vi "Sim_Update_Model.vi"(8 "dt (s)":dbl, 9 "State":T3, 10 "Settings":T4={"UI Update Interval (ms)"=200, "Max dt (s)"=1.0, "Initial SOC (%)"=50.0, "Rest Voltage (V)"=12.0, "Ambient Temperature (degC)"=25.0, "Voltage Time Constant (s)"=5.0, "Current Time Constant (s)"=1.0, "Thermal Time Constant (s)"=120.0, "Heating Coefficient (degC/s per A^2)"=0.002, "SOC Speed Factor"=1.0, "Charge Complete SOC (%)"=100.0, "Discharge Complete SOC (%)"=0.0, "Max Voltage Limit (V)"=15.0, "Max Current Limit (A)"=10.0, "Max Temperature Limit (degC)"=45.0, "Max C-Rate (1/h)"=5.0, "Max Duration (min)"=600.0, "History Length (samples)"=3000, "Inject E-Stop"=FALSE, "Inject Overvoltage"=FALSE, "Inject Overcurrent"=FALSE, "Inject Overtemperature"=FALSE}, 11 "Sim Data in":T1) -> (3 "Sim Data out":T1)   [LabVIEW 2019]
doc: "DEMONSTRATION MODEL - the replaceable sensor source. One simulation step of length dt. SOC: ideal C-rate integration (dSOC = C x 100 x dt x SpeedFactor / 3600) clamped 0..100. Voltage and current: first-order approach to the setpoints (discharge current negative). Temperature: current-squared heating with first-order cooling to ambient. OUTPUT INTERLOCK: only CHARGING enables the simulated supply and only DISCHARGING the simulated load; every other state forces both OFF and current to 0. Not an electrochemical battery model. A later hardware phase replaces this VI."
uses:
  Sim_Data.ctl
  Test_State_Enum2.ctl
  Sim_Settings.ctl
  Sim_State_Enum.ctl
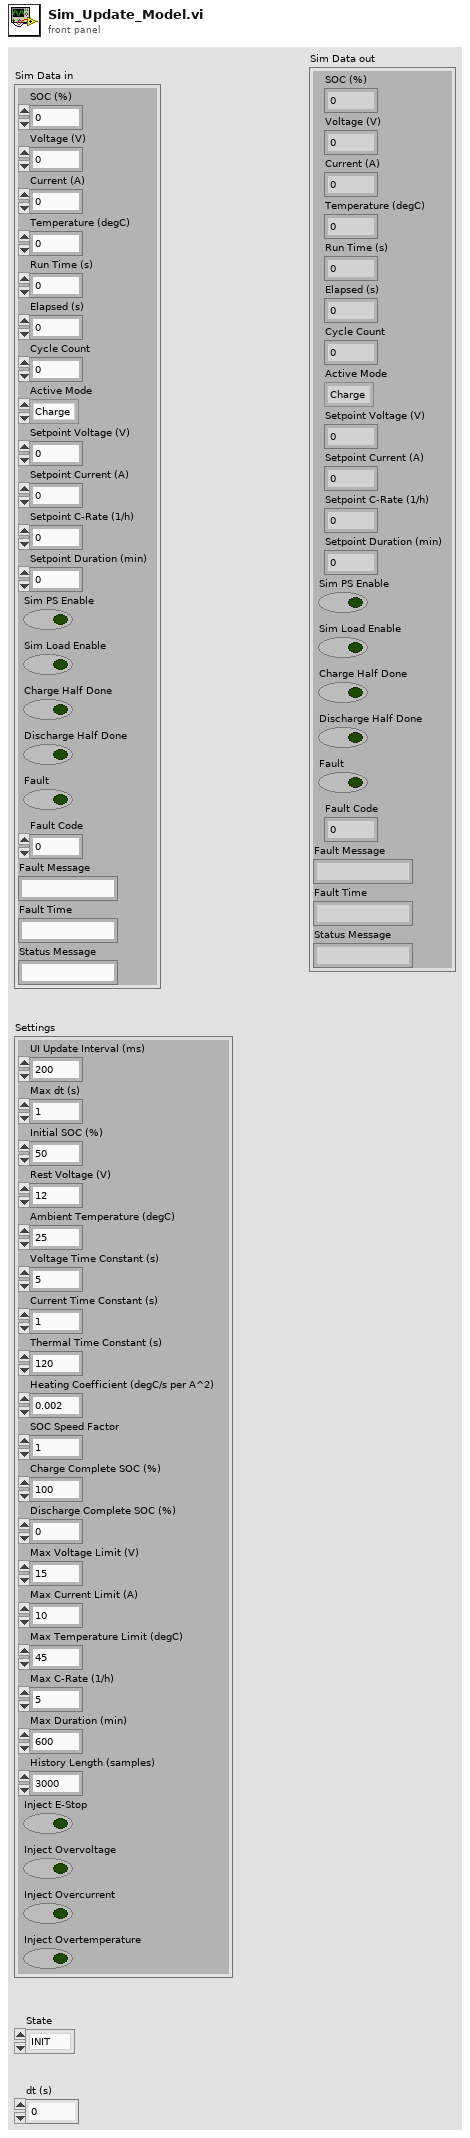
[diagram p1: front panel]
types:
  T1 = typedef "Sim_Data.ctl" = cluster{"SOC (%)":dbl, "Voltage (V)":dbl, "Current (A)":dbl, "Temperature (degC)":dbl, "Run Time (s)":dbl, "Elapsed (s)":dbl, "Cycle Count":u32, "Active Mode":T2, "Setpoint Voltage (V)":dbl, "Setpoint Current (A)":dbl, "Setpoint C-Rate (1/h)":dbl, "Setpoint Duration (min)":dbl, "Sim PS Enable":bool, "Sim Load Enable":bool, "Charge Half Done":bool, "Discharge Half Done":bool, "Fault":bool, "Fault Code":i32, "Fault Message":string, "Fault Time":string, "Status Message":string}
  T2 = typedef "Test_State_Enum2.ctl" = enum16{"Charge", "Discharge"}
  T3 = typedef "Sim_State_Enum.ctl" = enum16{"INIT", "IDLE", "CHARGING", "DISCHARGING", "STOPPED", "FAULT"}
  T4 = typedef "Sim_Settings.ctl" = cluster{"UI Update Interval (ms)":i32, "Max dt (s)":dbl, "Initial SOC (%)":dbl, "Rest Voltage (V)":dbl, "Ambient Temperature (degC)":dbl, "Voltage Time Constant (s)":dbl, "Current Time Constant (s)":dbl, "Thermal Time Constant (s)":dbl, "Heating Coefficient (degC/s per A^2)":dbl, "SOC Speed Factor":dbl, "Charge Complete SOC (%)":dbl, "Discharge Complete SOC (%)":dbl, "Max Voltage Limit (V)":dbl, "Max Current Limit (A)":dbl, "Max Temperature Limit (degC)":dbl, "Max C-Rate (1/h)":dbl, "Max Duration (min)":dbl, "History Length (samples)":i32, "Inject E-Stop":bool, "Inject Overvoltage":bool, "Inject Overcurrent":bool, "Inject Overtemperature":bool}
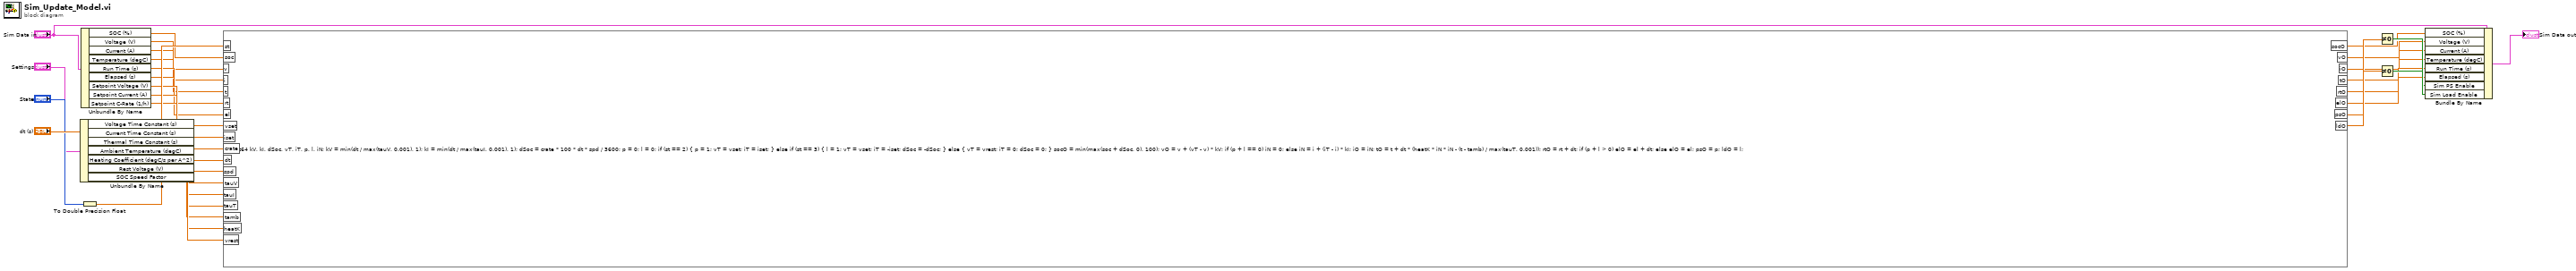
[diagram p0: block diagram]
diagram:
  n1 = Unbundle By Name("Settings") -> ("Voltage Time Constant (s)"=w15:dbl, "Current Time Constant (s)"=w16:dbl, "Thermal Time Constant (s)"=w17:dbl, "Ambient Temperature (degC)"=w18:dbl, "Heating Coefficient (degC/s per A^2)"=w19:dbl, "Rest Voltage (V)"=w20:dbl, "SOC Speed Factor"=w21:dbl)
  n2 = Unbundle By Name("Sim Data in") -> ("SOC (%)"=w6:dbl, "Voltage (V)"=w7:dbl, "Current (A)"=w8:dbl, "Temperature (degC)"=w9:dbl, "Run Time (s)"=w10:dbl, "Elapsed (s)"=w11:dbl, "Setpoint Voltage (V)"=w12:dbl, "Setpoint Current (A)"=w13:dbl, "Setpoint C-Rate (1/h)"=w14:dbl)
  n3 = To Double Precision Float(number="State") -> (double precision float=w22:dbl)
  n4 = formula code="float64 kV, kI, dSoc, vT, iT, p, l, iN; kV = min(dt / max(tauV, 0.001), 1); kI = min(dt / max(tauI, 0.001), 1); dSoc = crate * 100 * dt * spd / 3600; p = 0; l = 0; if (st == 2) { p = 1; vT = vset; iT = iset; } else if (st == 3) { l = 1; vT = vset; iT = -iset; dSoc = -dSoc; } else { vT = vrest; iT = 0; dSoc = 0; } socO = min(max(soc + dSoc, 0), 100); vO = v + (vT - v) * kV; if (p + l == 0) iN = 0; else iN = i + (iT - i) * kI; iO = iN; tO = t + dt * (heatK * iN * iN - (t - tamb) / max(tauT, 0.001)); rtO = rt + dt; if (p + l > 0) elO = el + dt; else elO = el; psO = p; ldO = l;"("st"=w22, "soc"=w6, "v"=w7, "i"=w8, "t"=w9, "rt"=w10, "el"=w11, "vset"=w12, "iset"=w13, "crate"=w14, "dt"="dt (s)", "spd"=w21, "tauV"=w15, "tauI"=w16, "tauT"=w17, "tamb"=w18, "heatK"=w19, "vrest"=w20) -> ("socO"=w23:dbl, "vO"=w24:dbl, "iO"=w25:dbl, "tO"=w26:dbl, "rtO"=w27:dbl, "elO"=w28:dbl, "psO"=w29:dbl, "ldO"=w30:dbl)
  n5 = Not Equal To 0?(x=w29) -> (x != 0?=w31:bool)
  n6 = Not Equal To 0?(x=w30) -> (x != 0?=w32:bool)
  n7 = Bundle By Name(cluster="Sim Data in", "SOC (%)"=w23, "Voltage (V)"=w24, "Current (A)"=w25, "Temperature (degC)"=w26, "Run Time (s)"=w27, "Elapsed (s)"=w28, "Sim PS Enable"=w31, "Sim Load Enable"=w32) -> (→"Sim Data out":T1)
